vi "Handle Response.vi"(7 "Processing In":refnum<class "Processing.lvclass">, 11 "Session Response Handler in":refnum<class "Session Response Handler.lvclass">) -> (0 "error out":errorcluster, 5 "Processing":refnum<class "Processing.lvclass">)   [LabVIEW 2020, in "HTTP Server.lvlib" / "Session Response Handler.lvclass"]
uses:
  Session Response Handler.lvclass
  Processing/Processing.lvclass
  Processing/Processing.lvclass/Processing.ctl
  lv-http-util/HTTP Utils/Cookie Attributes.ctl
  lv-http-util/HTTP Utils/Cookie SameSite.ctl
  lv-http-util/HTTP Utils/Cookie Prefix.ctl
  Session/Session.lvclass
  lv-http-util/HTTP Utils/Response/Response.lvclass
  lv-http-util/HTTP Utils/HTTP Utils.lvlib
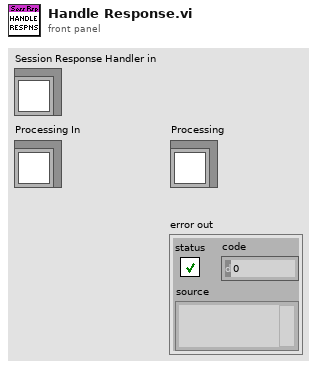
[diagram p1: front panel]
types:
  T1 = typedef "HTTP Utils.lvlib/Cookie Attributes.ctl" = cluster{"Expires":timestamp, "Secure":bool, "HttpOnly":bool, "Domain":string, "Path":string, "SameSite":T2, "Prefix":T3, "Max-Age Expiry":bool}
  T2 = typedef "HTTP Utils.lvlib/Cookie SameSite.ctl" = enum16{"Unset (Lax)", "Lax", "Strict", "None"}
  T3 = typedef "HTTP Utils.lvlib/Cookie Prefix.ctl" = enum16{"None", "Host", "Secure"}
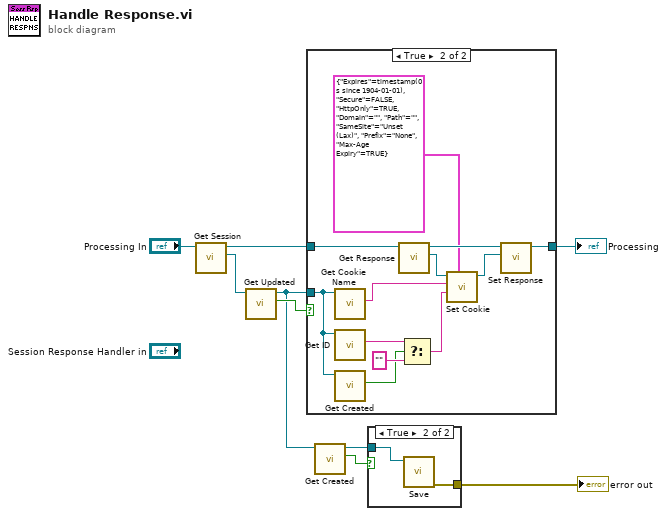
[diagram p0: block diagram]
diagram:
  n1 = call "Get Session.vi"("Processing in"="Processing In") -> ("Session"=w3:refnum<class "Session.lvclass">, "Processing out"=w2:refnum<class "Processing.lvclass">)  [unwired: 9 in]
  n2 = call "Get Updated.vi"("Session in"=w3) -> ("Updated"=w9:bool, "Session out"=w6:refnum<class "Session.lvclass">)  [unwired: 8 in, 1 out]
  n3 = case shown="True" w9 {
    tunnel: w6 -> [_ w21]
    tunnel: [w10 w14] -> w8
    tunnel: w2 -> [w10 w13]
    frame False {
    }
    frame True {
      n4 = call "Get Cookie Name.vi"("Session in"=w21) -> ("Cookie Name"=w22:string)  [unwired: 8 in, 2 out]
      n5 = call "Get ID.vi"("Session in"=w21) -> ("ID"=w20:string)  [unwired: 8 in, 2 out]
      n6 = call "Get Created.vi"("Session in"=w21) -> ("Created"=w18:bool)  [unwired: 8 in, 2 out]
      n7 = call "Get Response.vi"("Processing in"=w13) -> ("Response"=w16:refnum<class "Response.lvclass">, "Processing out"=w15:refnum<class "Processing.lvclass">)  [unwired: 9 in]
      n8 = Select(t=w20, s=w18, f="") -> (s? t:f=w17:string)
      n9 = call "Set Cookie.vi"("Attributes (HttpOnly)"=T1 {"Expires"=timestamp(0 s since 1904-01-01), "Secure"=FALSE, "HttpOnly"=TRUE, "Domain"="", "Path"="", "SameSite"=enum."Unset (Lax)", "Prefix"=enum."None", "Max-Age Expiry"=TRUE}, "Value"=w17, "Name"=w22, "Response in"=w16) -> ("Response out"=w12:refnum<class "Response.lvclass">)  [unwired: 6 in, 1 out]
      n10 = call "Set Response.vi"("Response"=w12, "Processing in"=w15) -> ("Processing out"=w14:refnum<class "Processing.lvclass">)  [unwired: 9 in]
    }
  }
  "Processing" <- w8
  n11 = call "Get Created.vi"("Session in"=w6) -> ("Created"=w5:bool, "Session out"=w4:refnum<class "Session.lvclass">)  [unwired: 8 in, 1 out]
  n12 = case shown="True" w5 {
    tunnel: [_ w24] -> w7
    tunnel: w4 -> [_ w23]
    frame False {
    }
    frame True {
      n13 = call "Save.vi"("Session in"=w23) -> ("error out"=w24:errorcluster)  [unwired: 9 in, 1 out]
    }
  }
  "error out" <- w7
